vi "Axis_Cmd.vi"(8 "error in (no error)":errorcluster, 10 "Command":string, 11 "VISA Refnum name":refnum<visa-resource-name>) -> (0 "error out":errorcluster, 2 "read buffer":string, 3 "VISA Refnum name out":refnum<visa-resource-name>)   [LabVIEW 2018]
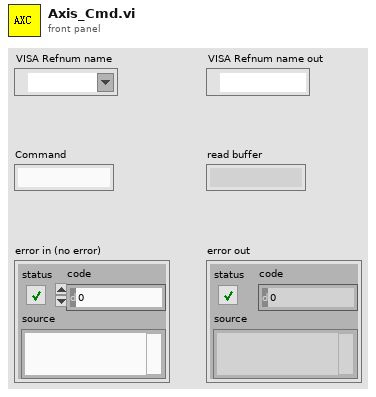
[diagram p1: front panel]
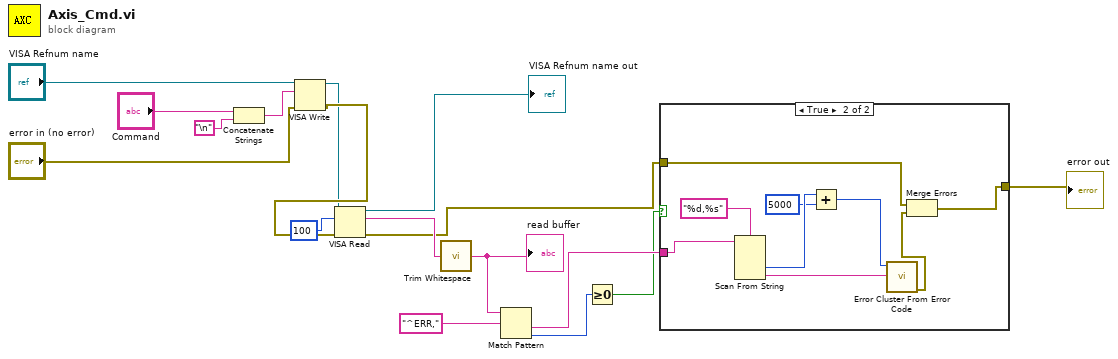
[diagram p0: block diagram]
diagram:
  n1 = Concatenate Strings("Command", "\n") -> (w12:string)
  n2 = VISA Write(VISA resource name="VISA Refnum name", write buffer=w12, error in (no error)="error in (no error)") -> (VISA resource name out=w14:refnum<visa-resource-name>, error out=w16:errorcluster)  [unwired: 1 out]
  n3 = VISA Read(VISA resource name=w14, byte count=u32 100, error in (no error)=w16) -> (VISA resource name out=→"VISA Refnum name out":refnum<visa-resource-name>, read buffer=w8:string, error out=w5:errorcluster)  [unwired: 1 out]
  n4 = call-poly <vilib>:"Trim Whitespace.vi"("string"=w8) -> ("trimmed string"=w7:string)  [unwired: 1 in]
  "read buffer" <- w7
  n5 = Match Pattern(string=w7, regular expression="^ERR,") -> (after substring=w4:string, offset past match=w2:i32)  [unwired: 1 in, 2 out]
  n6 = Greater Or Equal To 0?(x=w2) -> (x >= 0?=w1:bool)
  n7 = case shown="True" w1 {
    tunnel: w5 -> [w18 w21]
    tunnel: w4 -> [_ w27]
    tunnel: [w18 w19] -> w3
    frame False {
    }
    frame True {
      n8 = Scan From String(format string="%d,%s", input string=w27) -> (output 1=w25:i32, output 2=w22:string)  [unwired: 4 in, 3 out]
      n9 = Add(x=w25, y=5000) -> (x+y=w23:i32)
      n10 = call <vilib>:"Error Cluster From Error Code.vi"("error message (\"\")"=w22, "error code (0)"=w23) -> ("error out"=w20:errorcluster)  [unwired: 7 in]
      n11 = Merge Errors(w21, w20) -> (w19:errorcluster)
    }
  }
  "error out" <- w3
